vi "CIPC L2Enet FIFO.vi"() -> (3 "CIF_CIPC_L2Enet.lvclass":refnum<class "CIF_Iceoryx_L2Enet.lvclass">)   [LabVIEW 2021, in "CIF_Iceoryx_L2Enet.lvclass"]
uses:
  CIF_Iceoryx_L2Enet.lvclass
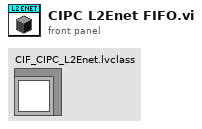
[diagram p1: front panel]
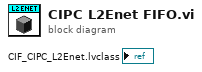
[diagram p0: block diagram]
diagram:
